vi "Set Icon.vi"(8 "error in":errorcluster, 11 "ILabVIEWFile in":refnum<class "LabVIEW File.lvclass">) -> (0 "error out":errorcluster, 3 "ILabVIEWFile out":refnum<class "LabVIEW File.lvclass">)   [LabVIEW 2026, in "LabVIEW File.lvclass"]
doc: "Set VI (or control) text icon using the name of the file from class private data."
uses:
  LabVIEW File.lvclass
  LabVIEW File.lvclass/LabVIEW File.ctl
  <vilib>/LabVIEW Icon API/Set Text Icon/Text-Based VI Icon.lvlib
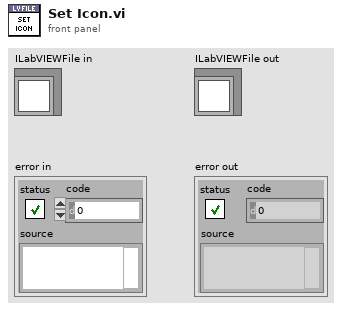
[diagram p1: front panel]
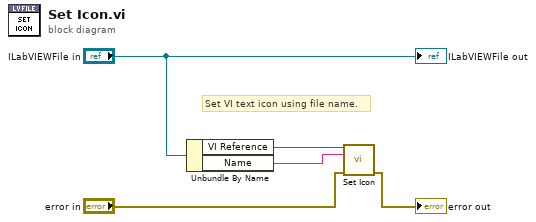
[diagram p0: block diagram]
diagram:
  # "Set VI text icon using file name."
  n1 = Unbundle By Name("ILabVIEWFile in") -> ("VI Reference"=w1:refnum<vi>, "Name"=w2:string)
  n2 = call <vilib>:"Set Icon.vi"("VI"=w1, "user-supplied text (\"\" - use VI file name)"=w2, "error in"="error in") -> ("error out"=→"error out":errorcluster)  [unwired: 11 in, 1 out]
  "ILabVIEWFile out" <- "ILabVIEWFile in"
